vi "Update Mock Class.vi"(8 "error in (no error)":errorcluster, 10 "Mock Class Path":path=path "C:/Users/AntonSundqvist/Desktop/New folder/test.lvclass") -> (0 "error out":errorcluster)   [LabVIEW 2020, in "Mock Class Updater.lvclass"]
uses:
  Mock Class Updater.lvclass
  Mock Class Updater.lvclass/Mock Class Updater.ctl
  Mock Class Generator/Mock Class Generator.lvclass
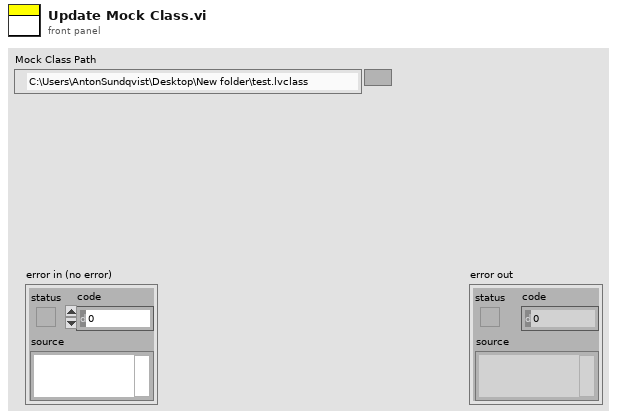
[diagram p1: front panel]
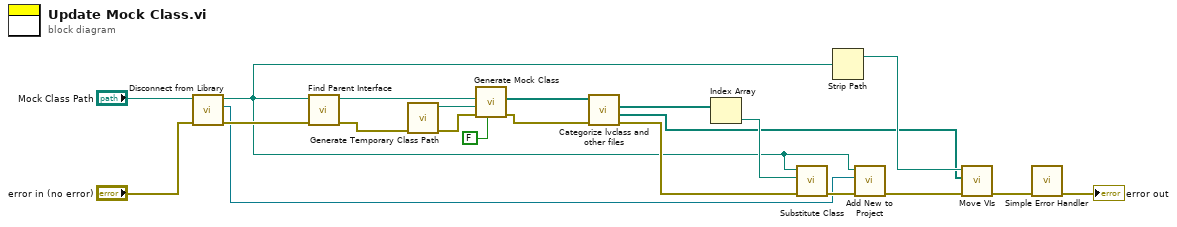
[diagram p0: block diagram]
diagram:
  n1 = call "Disconnect from Library.vi"("error in (no error)"="error in (no error)", "Mock Class Path"="Mock Class Path") -> ("error out"=w4:errorcluster, "Owning Library"=w1:refnum<vi>, "Mock Class Path Out"=w2:path)  [unwired: 7 in]
  n2 = call "Find Parent Interface.vi"("error in (no error)"=w4, "Mock Class Path"=w2) -> ("error out"=w19:errorcluster, "Parent Interface"=w20:path)  [unwired: 8 in]
  n3 = call "Generate Temporary Class Path.vi"("error in (no error)"=w19) -> ("error out"=w10:errorcluster, "appended path"=w9:path)  [unwired: 9 in]
  n4 = call "Generate Mock Class.vi"("Add to lvproj?"=FALSE, "error in (no error)"=w10, "Destination Class Path"=w9, "Source Class Path"=w20) -> ("error out"=w16:errorcluster, "Created Files"=w17:path[])  [unwired: 6 in]
  n5 = call "Categorize lvclass and other files.vi"("error in (no error)"=w16, "Created Files"=w17) -> ("error out"=w15:errorcluster, "Other Files"=w6:path[], "LVClass Files"=w14:path[])  [unwired: 7 in]
  n6 = Index Array(array=w14) -> (element=w7:path)  [unwired: 1 in]
  n7 = call "Substitute Class.vi"("error in (no error)"=w15, "New Class"=w7, "Class to Replace"=w2) -> ("error out"=w13:errorcluster)  [unwired: 8 in]
  n8 = Strip Path(path=w2) -> (stripped path=w11:path)  [unwired: 1 out]
  n9 = call "Add New to Project.vi"("error in (no error)"=w13, "Owning Library"=w1, "Path"=w2) -> ("error out"=w8:errorcluster)  [unwired: 8 in]
  n10 = call "Move VIs.vi"("error in (no error)"=w8, "VIs to Move"=w6, "Destination"=w11) -> ("error out"=w12:errorcluster)  [unwired: 8 in]
  n11 = call <vilib>:"Simple Error Handler.vi"("error in (no error)"=w12) -> ("error out"=→"error out":errorcluster)  [unwired: 4 in, 4 out]
